vi "UpdateCommandWrapperReferencesMac.vi"() -> ()   [LabVIEW 2026]
doc: "Bordeaux: rewrites the managed command wrapper references VI in the robot target context. Deletes its Static VI References, adds one per wrapper path, records the description and saves. Refuses an unmarked VI (5001), unsaved edits (5002) and an unknown target (5003). Never runs a wrapper."
uses:
  <vilib>/Utility/traverseref.llb/VI Scripting - Traverse.lvlib
  <vilib>/Utility/traverseref.llb/TRef TravTarget.ctl
  <vilib>/Utility/miscctls.llb/LVPointTypeDef.ctl
panel:
  out "error out":errorcluster
  out "reference count":i32
  out "previous description":string
  out "context name":string
  in  "wrapper paths":string[](array[string])
  in  "marker":string
  in  "description":string
  in  "references path":string
  in  "target name":string
  in  "project path":string
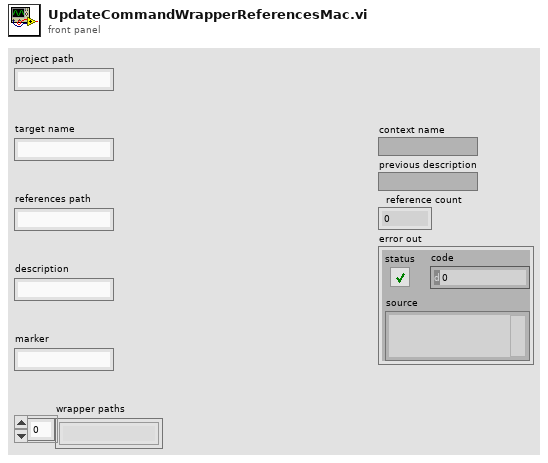
[diagram p1: front panel]
types:
  T1 = typedef "TRef TravTarget.ctl" = enum16{"FP", "BD", "Other"}
  T2 = typedef "LVPointTypeDef.ctl" = cluster{"Horizontal":i16, "Vertical":i16}
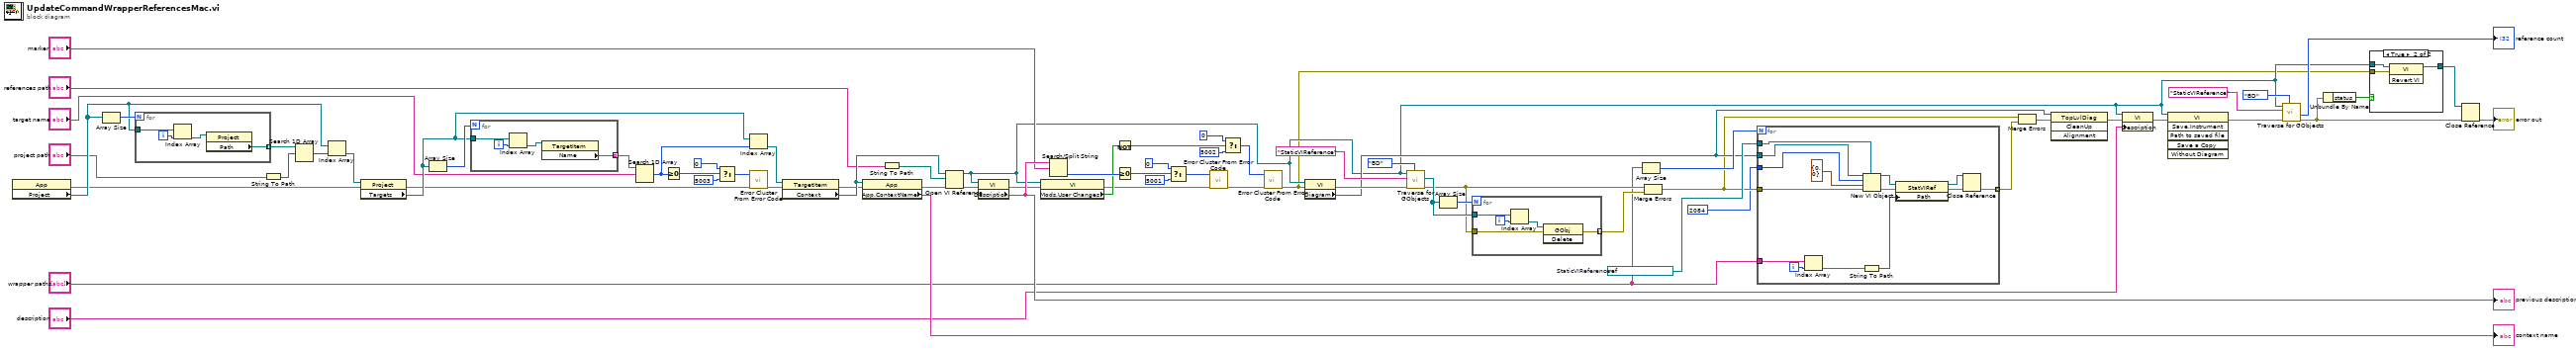
[diagram p0: block diagram]
diagram:
  w19 = refnum<vi> refnum  # StaticVIReference
  n1 = property class="App"() -> (error out=w63:errorcluster, "Project"=w69:refnum<vi>[])  [unwired: 2 in, 1 out]
  n2 = Array Size(array=w69) -> (size(s)=w70:i32)
  n3 = for {
    N: w70 -> [_]
    tunnel: w69 -> [w74]
    tunnel: [w71] -> w66 mode=indexing
    i -> [w73]
    n4 = Index Array(array=w74, index=w73) -> (element=w72:refnum<vi>)
    n5 = property class="Project"(reference=w72) -> ("Path"=w71:path)  [unwired: 1 in, 2 out]
  }
  n6 = String To Path(string="project path") -> (path=w67:path)
  n7 = Search 1D Array(1D array=w66, element=w67) -> (index of element=w65:i32)  [unwired: 1 in]
  n8 = Index Array(array=w69, index=w65) -> (element=w64:refnum<vi>)
  n9 = property class="Project"(reference=w64, error in=w63) -> (error out=w53:errorcluster, "Targets"=w61:refnum<vi>[])  [unwired: 1 out]
  n10 = Array Size(array=w61) -> (size(s)=w62:i32)
  n11 = for {
    N: w62 -> [_]
    tunnel: w61 -> [w78]
    tunnel: [w75] -> w59 mode=indexing
    i -> [w77]
    n12 = Index Array(array=w78, index=w77) -> (element=w76:refnum<vi>)
    n13 = property class="TargetItem"(reference=w76) -> ("Name"=w75:string)  [unwired: 1 in, 2 out]
  }
  n14 = Search 1D Array(1D array=w59, element="target name") -> (index of element=w58:i32)  [unwired: 1 in]
  n15 = Greater Or Equal To 0?(x=w58) -> (x >= 0?=w57:bool)
  n16 = Select(t=0, s=w57, f=5003) -> (s? t:f=w54:i32)
  n17 = Index Array(array=w61, index=w58) -> (element=w52:refnum<vi>)
  n18 = call <vilib>:"Error Cluster From Error Code.vi"("error in (no error)"=w53, "error code (0)"=w54) -> ("error out"=w51:errorcluster)  [unwired: 7 in]
  n19 = property class="TargetItem"(reference=w52, error in=w51) -> (error out=w49:errorcluster, "Context"=w50:refnum<vi>)  [unwired: 1 out]
  n20 = property class="App"(reference=w50, error in=w49) -> (error out=w45:errorcluster, "App.ContextName"=→"context name":string)  [unwired: 1 out]
  n21 = String To Path(string="references path") -> (path=w46:path)
  n22 = Open VI Reference(application reference (local)=w50, vi path=w46, error in (no error)=w45) -> (vi reference=w4:refnum<vi>, error out=w44:errorcluster)  [unwired: 3 in]
  n23 = property class="VI"(reference=w4, error in=w44) -> (error out=w40:errorcluster, "Description"=w43:string)  [unwired: 1 out]
  "previous description" <- w43
  n24 = property class="VI"(reference=w4, error in=w40) -> (error out=w34:errorcluster, "Mods.User Changes"=w39:bool)  [unwired: 1 out]
  n25 = Search/Split String(string=w43, search string/char (-)="marker") -> (offset of match=w41:i32)  [unwired: 1 in, 2 out]
  n26 = Not(x=w39) -> (.not. x?=w33:bool)
  n27 = Greater Or Equal To 0?(x=w41) -> (x >= 0?=w38:bool)
  n28 = Select(t=0, s=w38, f=5001) -> (s? t:f=w35:i32)
  n29 = call <vilib>:"Error Cluster From Error Code.vi"("error in (no error)"=w34, "error code (0)"=w35) -> ("error out"=w29:errorcluster)  [unwired: 7 in]
  n30 = Select(t=0, s=w33, f=5002) -> (s? t:f=w30:i32)
  n31 = call <vilib>:"Error Cluster From Error Code.vi"("error in (no error)"=w29, "error code (0)"=w30) -> ("error out"=w3:errorcluster)  [unwired: 7 in]
  n32 = property class="VI"(reference=w4, error in=w3) -> (error out=w27:errorcluster, "Diagram"=w18:refnum<vi>)  [unwired: 1 out]
  n33 = call <vilib>:"Traverse for GObjects.vi"("Traverse Target"=TRef_TravTarget."BD", "error in (no error)"=w27, "Class Name"="StaticVIReference", "VI Refnum"=w4) -> ("error out"=w23:errorcluster, "References"=w24:refnum<vi>[])  [unwired: 4 in, 2 out]
  n34 = Array Size(array=w24) -> (size(s)=w25:i32)
  n35 = for {
    N: w25 -> [_]
    tunnel: w24 -> [w83]
    tunnel: w23 -> [w80]
    tunnel: [w79] -> w22 mode=indexing
    i -> [w82]
    n36 = Index Array(array=w83, index=w82) -> (element=w81:refnum<vi>)
    n37 = invoke class="GObj" method="Delete"(reference=w81, error in=w80) -> (error out=w79:errorcluster)  [unwired: 1 in, 2 out]
  }
  n38 = Array Size(array="wrapper paths") -> (size(s)=w21:i32)
  n39 = Merge Errors(w23, w22) -> (w17:errorcluster)
  n40 = for {
    N: w21 -> [_]
    tunnel: "wrapper paths" -> [w97]
    tunnel: w19 -> [w95]
    tunnel: w18 -> [w94]
    tunnel: w17 -> [w93]
    tunnel: u32 2084 -> [w92]
    tunnel: [w84] -> w15 mode=indexing
    i -> [w96]
    n41 = Index Array(array=w97, index=w96) -> (element=w90:string)
    n42 = String To Path(string=w90) -> (path=w87:path)
    n43 = New VI Object(vi object class=w95, owner refnum=w94, style=w92, position/next to=T2 {"Horizontal"=0, "Vertical"=0} ("location"), 8:w93) -> (object refnum=w89:refnum<vi>, 0:w88:errorcluster)  [unwired: 3 in]
    n44 = property class="StatVIRef"(reference=w89, error in=w88, "Path"=w87) -> (reference out=w86:refnum<vi>, error out=w85:errorcluster)
    n45 = Close Reference(reference=w86, error in (no error)=w85) -> (error out=w84:errorcluster)
  }
  n46 = Merge Errors(w17, w15) -> (w14:errorcluster)
  n47 = invoke class="TopLvlDiag" method="CleanUp"(reference=w18, error in=w14) -> (error out=w13:errorcluster)  [unwired: 2 in, 3 out]
  n48 = property class="VI"(reference=w4, error in=w13, "Description"="description") -> (error out=w11:errorcluster)  [unwired: 1 out]
  n49 = invoke class="VI" method="Save.Instrument"(reference=w4, error in=w11) -> (error out=w9:errorcluster)  [unwired: 4 in, 5 out]
  n50 = call <vilib>:"Traverse for GObjects.vi"("Traverse Target"=TRef_TravTarget."BD", "error in (no error)"=w9, "Class Name"="StaticVIReference", "VI Refnum"=w4) -> ("error out"=w6:errorcluster, "# of Refs"=→"reference count":i32)  [unwired: 4 in, 2 out]
  n51 = Unbundle By Name(w6) -> ("status"=w5:bool)
  n52 = case shown="True" w5 {
    tunnel: w4 -> [w98 w101]
    tunnel: w3 -> [_ w100]
    tunnel: [w98 w99] -> w2
    frame False {
    }
    frame True {
      n53 = invoke class="VI" method="Revert VI"(reference=w101, error in=w100) -> (reference out=w99:refnum<vi>)  [unwired: 1 in, 2 out]
    }
  }
  n54 = Close Reference(reference=w2, error in (no error)=w6) -> (error out=→"error out":errorcluster)
